vi "Image.vi"(2 "XRef":refnum<vi>, 3 "State In":T1) -> (0 "Image":picture)   [LabVIEW 2012, in "OpenG FilterArray.xnode"]
uses:
  OpenG FilterArray.xnode
  State.ctl
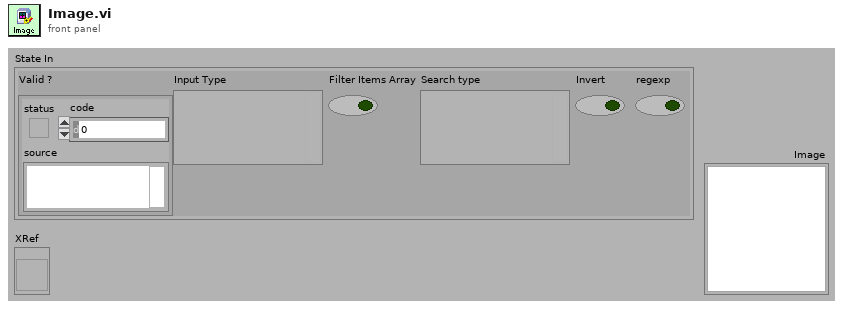
[diagram p1: front panel]
types:
  T1 = typedef "OpenG FilterArray.xnode/State.ctl" = cluster{"Valid ?":errorcluster, "Input Type":variant, "Filter Items Array":bool, "Search type":variant, "Invert":bool, "regexp":bool}
  T2 = typedef "imagedata.ctl" = cluster{"image type":i32, "image depth":i32, "image":u8[], "mask":u8[], "colors":u32[], "Rectangle":cluster{"left":i16, "top":i16, "right":i16, "bottom":i16}}
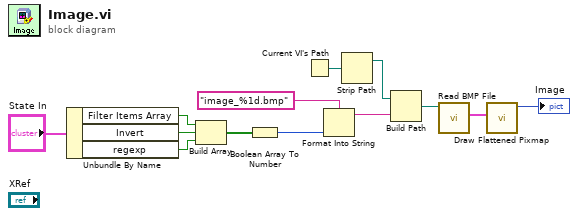
[diagram p0: block diagram]
diagram:
  n1 = Unbundle By Name("State In") -> ("Filter Items Array"=w7:bool, "Invert"=w6:bool, "regexp"=w5:bool)
  n2 = Build Array(w7, w6, w5) -> (w4:bool[])
  n3 = Boolean Array To Number(Boolean array=w4) -> (number=w2:u32)
  n4 = Current VI's Path() -> (path=w13:path)
  n5 = Format Into String(format string="image_%1d.bmp" ("name or relative path"), w2) -> (resulting string=w1:string)  [unwired: 2 in, 1 out]
  n6 = Strip Path(path=w13) -> (stripped path=w12:path)  [unwired: 1 out]
  n7 = Build Path(base path=w12, name or relative path=w1) -> (appended path=w11:path)
  n8 = call <vilib>:"Read BMP File.vi"("path to BMP file"=w11) -> ("image data"=w10:T2)  [unwired: 1 in, 9 out]
  n9 = call <vilib>:"Draw Flattened Pixmap.vi"("image data"=w10) -> ("new picture"=→"Image":picture)  [unwired: 1 in, 7 out]
